vi "RemoteVI Fixture Value Line.vi"(0 "label":string, 5 "value":string, 11 "error in":errorcluster) -> (4 "line":string, 15 "error out":errorcluster)   [LabVIEW 2020]
doc: "Event-log helper of RemoteVI Fixture.vi. Builds one value line of the log: value TAB label TAB value LF, with every line feed inside value written as the two characters \\n so the line stays one line. error in is passed through unchanged."
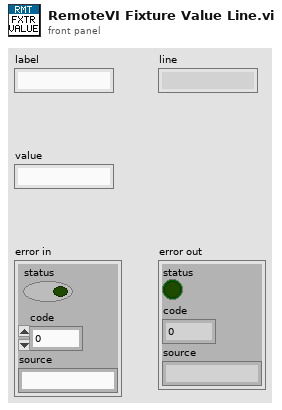
[diagram p1: front panel]
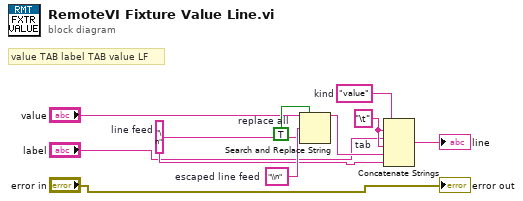
[diagram p0: block diagram]
diagram:
  w8 = TRUE  # replace all
  w7 = "\\n"  # escaped line feed
  w6 = "\n"  # line feed
  w5 = "\t"  # tab
  w4 = "value"  # kind
  # "value TAB label TAB value LF"
  n1 = Search and Replace String(replace all?=w8, input string="value", search string=w6, replace string=w7) -> (result string=w9:string)  [unwired: 4 in, 3 out]
  n2 = Concatenate Strings(w4, w5, "label", w5, w9, w6) -> (→"line":string)
  "error out" <- "error in"
